vi "Parse QD Text.vi"(10 "Shift Pressed?":bool, 11 "QD Combo Box Text":string) -> (2 "Parameter":string, 3 "Command":T1=enum."Run")   [LabVIEW 2020]
doc: "Parse the QD Combo Box Text to interpret the command into an ENUM and pull out the paramters."
uses:
  Command Enum.ctl
panel:
  out "Parameters":string[](array[string])
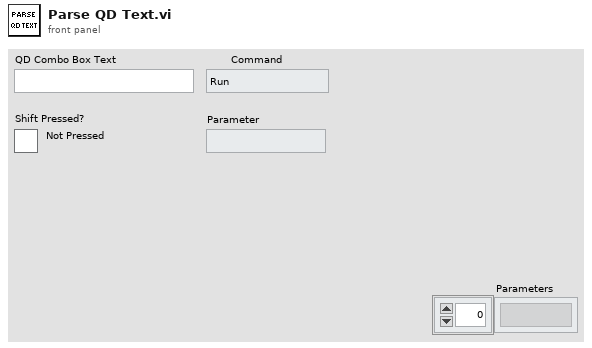
[diagram p1: front panel]
types:
  T1 = typedef "Command Enum.ctl" = enum16{"Invalid", "Invalid Alias", "Run", "Set", "Open", "Read", "Remove"}
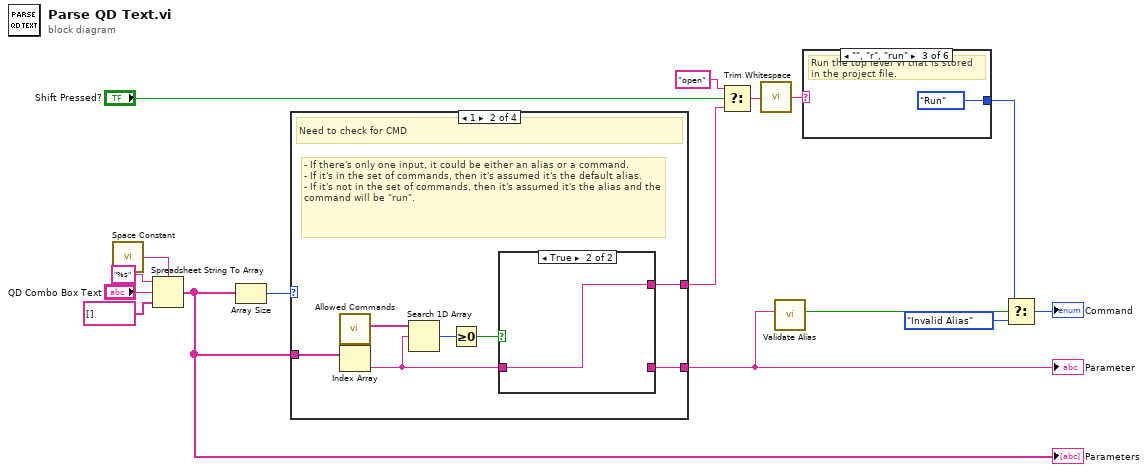
[diagram p0: block diagram]
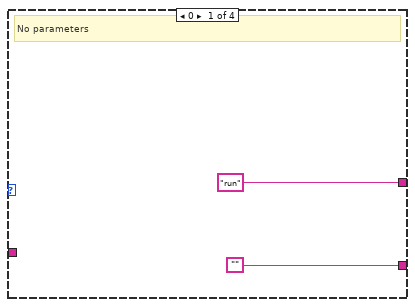
[diagram p2: hidden frame]
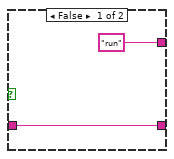
[diagram p3: hidden frame]
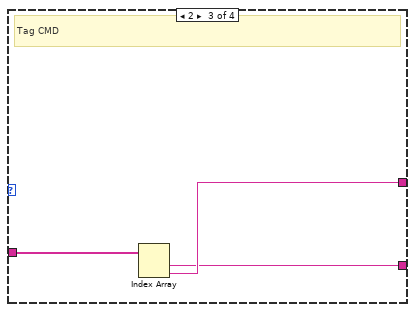
[diagram p4: hidden frame]
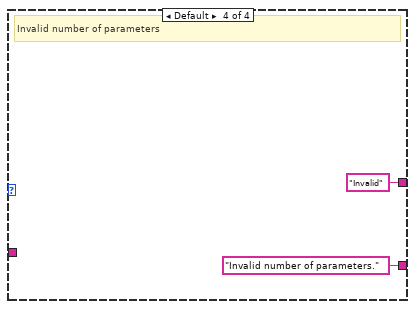
[diagram p5: hidden frame]
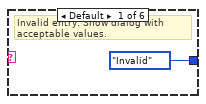
[diagram p6: hidden frame]
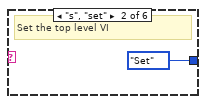
[diagram p7: hidden frame]
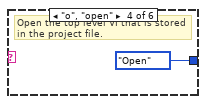
[diagram p8: hidden frame]
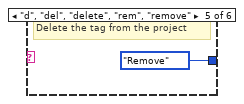
[diagram p9: hidden frame]
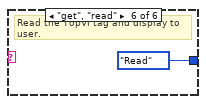
[diagram p10: hidden frame]
diagram:
  n1 = call <vilib>:"Space Constant.vi"() -> ("String"=w12:string)
  n2 = Spreadsheet String To Array(delimiter (Tab)=w12, format string="%s", spreadsheet string="QD Combo Box Text", array type (2D Dbl)=string[] []) -> (array=w6:string[])
  "Parameters" <- w6
  n3 = Array Size(array=w6) -> (size(s)=w9:i32)
  n4 = case shown="1" w9 {
    tunnel: ["run" w20 w30 "Invalid"] -> w7
    tunnel: w6 -> [_ w24 w31 _]
    tunnel: ["" w19 w29 "Invalid number of parameters."] -> w5
    frame 0 {
      # "No parameters"
    }
    frame 1 {
      # "- If there's only one input, it could be either an alias or a command.\n- If it's in the set of commands, then it's assumed it's the default alias.\n- If it's not in the set of commands, then it's assumed it's the alias and the command will be \"run\"."
      # "Need to check for CMD"
      n5 = call "Allowed Commands.vi"() -> ("Allowed Commands"=w25:string[])  [unwired: 11 in]
      n6 = Index Array(array=w24) -> (element=w21:string)  [unwired: 1 in]
      n7 = Search 1D Array(1D array=w25, element=w21) -> (index of element=w23:i32)  [unwired: 1 in]
      n8 = Greater Or Equal To 0?(x=w23) -> (x >= 0?=w22:bool)
      n9 = case shown="True" w22 {
        tunnel: w21 -> [w27 w28]
        tunnel: ["run" w28] -> w20
        tunnel: [w27 _] -> w19
        frame False {
        }
        frame True {
        }
      }
    }
    frame 2 {
      # "Tag CMD"
      n10 = Index Array(array=w31) -> (element #1=w29:string, element #2=w30:string)  [unwired: 2 in]
    }
    frame Default {
      # "Invalid number of parameters"
    }
  }
  "Parameter" <- w5
  n11 = Select(t="open", s="Shift Pressed?", f=w7) -> (s? t:f=w16:string)
  n12 = call <vilib>:"Trim Whitespace.vi"("string"=w16) -> ("trimmed string"=w13:string)  [unwired: 1 in]
  n13 = call "Validate Alias.vi"("Alias"=w5) -> ("Valid Alias"=w4:bool)  [unwired: 10 in]
  n14 = case shown="\"\", \"r\", \"run\"" w13 {
    tunnel: [Command_Enum."Invalid" ("Command") Command_Enum."Set" ("Command") Command_Enum."Run" ("Command") Command_Enum."Open" ("Command") Command_Enum."Remove" ("Command") Command_Enum."Read" ("Command")] -> w1
    frame Default {
      # "Invalid entry. Show dialog with acceptable values."
    }
    frame "s", "set" {
      # "Set the top level VI"
    }
    frame "", "r", "run" {
      # "Run the top level VI that is stored in the project file."
    }
    frame "o", "open" {
      # "Open the top level VI that is stored in the project file."
    }
    frame "d", "del", "delete", "rem", "remove" {
      # "Delete the tag from the project"
    }
    frame "get", "read" {
      # "Read the TopVI tag and display to user."
    }
  }
  n15 = Select(t=w1, s=w4, f=Command_Enum."Invalid Alias") -> (s? t:f=→"Command":T1)
